vi "Test Project and Task Lists.vi"(8 "error in":errorcluster, 10 "Work Folder":path, 11 "Test Data Folder":path) -> (0 "error out":errorcluster, 2 "Report":string, 3 "Passed":bool)   [LabVIEW 2026]
doc: "Tests Project List.vi and Task List.vi on the schema-v2 sample data (Test Data\\Samples, copied into a new case folder and opened with Initialize Stores.vi). Checks: the active projects come in Sort Order with the inactive Internal left out; the project IDs are parallel to the names; the tasks of TimeTracker and of Client Website in Sort Order with the inactive Testing left out; the task named Development has a different ID in each project; an empty and an unknown Project ID give empty lists and no error.\n\nInputs: Test Data Folder (Tests\\Storage\\Test Data); Work Folder (each run works in a new case folder under it); error in. Outputs: Passed (every check passed and no error); Report (one PASS/FAIL line per check); error out.\n\nGenerated by: Claude"
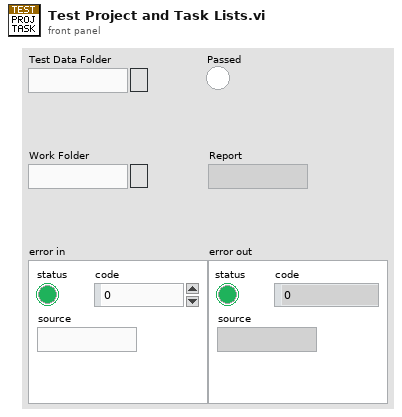
[diagram p1: front panel]
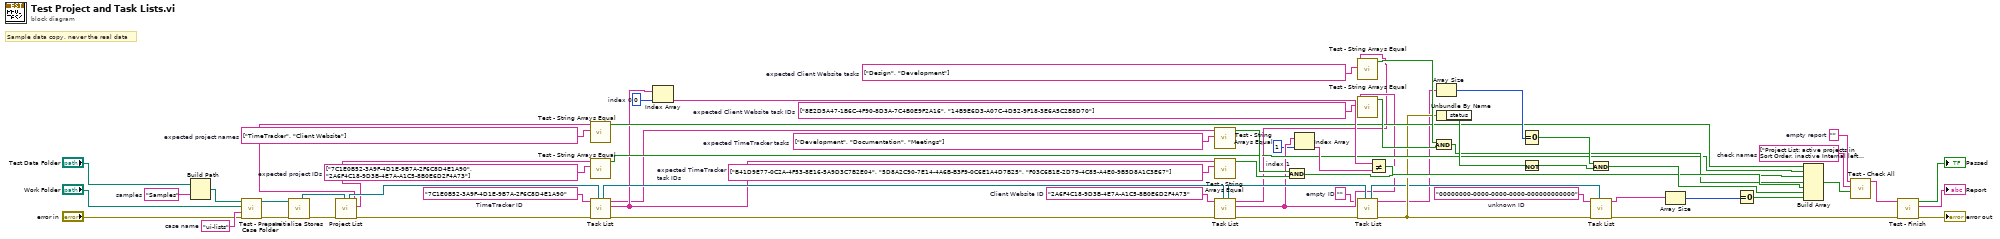
[diagram p0: block diagram]
diagram:
  w62 = string[] ["Project List: active projects in Sort Order, inactive Internal left out", "Project List: Project IDs parallel to the names", "Task List: TimeTracker tasks in Sort Order with their IDs", "Task List: Client Website tasks, inactive Testing left out, with their IDs", "Task List: Development has a different ID in each project", "Task List: empty Project ID gives an empty list and no error", "Task List: unknown Project ID gives an empty list"]  # check names
  w21 = 1  # index 1
  w20 = 0  # index 0
  w19 = string[] ["8E2D5A47-1B6C-4F90-8D3A-7C4B0E9F2A16", "14B9E6D3-A07C-4D52-9F18-3E6A5C2B8D70"]  # expected Client Website task IDs
  w18 = string[] ["Design", "Development"]  # expected Client Website tasks
  w17 = string[] ["B41D9E77-0C2A-4F53-8E16-5A9D3C7B2E04", "5D8A2C90-7E14-4A6B-B3F9-0C6E1A4D7B25", "F03C6B1E-2D79-4C85-A4E0-9B5D8A1C3E67"]  # expected TimeTracker task IDs
  w16 = string[] ["Development", "Documentation", "Meetings"]  # expected TimeTracker tasks
  w15 = string[] ["7C1E0B52-3A9F-4D1E-9B7A-2F6C8D4E1A90", "2A6F4C18-9D3B-4E7A-A1C5-8B0E6D2F4A73"]  # expected project IDs
  w14 = string[] ["TimeTracker", "Client Website"]  # expected project names
  w13 = "00000000-0000-0000-0000-000000000000"  # unknown ID
  w12 = ""  # empty ID
  w11 = "2A6F4C18-9D3B-4E7A-A1C5-8B0E6D2F4A73"  # Client Website ID
  w10 = "7C1E0B52-3A9F-4D1E-9B7A-2F6C8D4E1A90"  # TimeTracker ID
  w9 = ""  # empty report
  w8 = "ui-lists"  # case name
  w7 = "Samples"  # samples
  # "Sample data copy, never the real data"
  n1 = Build Path(base path="Test Data Folder", name or relative path=w7) -> (appended path=w22:path)
  n2 = call "Test - Prepare Case Folder.vi"("error in (no error)"="error in", "Case Name"=w8, "Work Folder"="Work Folder", "Source Folder"=w22) -> ("error out"=w24:errorcluster, "Case Folder"=w23:path)  [unwired: 6 in]
  n3 = call "Initialize Stores.vi"("error in"=w24, "Data Folder"=w23) -> ("error out"=w26:errorcluster, "Project Store out"=w25:refnum<class "Project Store.lvclass">)  [unwired: 5 in, 3 out]
  n4 = call "Project List.vi"("Project Store in"=w25, "error in"=w26) -> ("error out"=w30:errorcluster, "Project IDs"=w28:string[], "Project Names"=w27:string[], "Project Store out"=w29:refnum<class "Project Store.lvclass">)  [unwired: 6 in]
  n5 = call "Test - String Arrays Equal.vi"("Expected"=w14, "Actual"=w27) -> ("Equal?"=w44:bool)  [unwired: 8 in, 1 out]
  n6 = call "Test - String Arrays Equal.vi"("Expected"=w15, "Actual"=w28) -> ("Equal?"=w45:bool)  [unwired: 8 in, 1 out]
  n7 = call "Task List.vi"("Project Store in"=w29, "error in"=w30, "Project ID"=w10) -> ("error out"=w34:errorcluster, "Task IDs"=w32:string[], "Task Names"=w31:string[], "Project Store out"=w33:refnum<class "Project Store.lvclass">)  [unwired: 5 in]
  n8 = Index Array(array=w32, index=w20) -> (element=w52:string)
  n9 = call "Test - String Arrays Equal.vi"("Expected"=w16, "Actual"=w31) -> ("Equal?"=w46:bool)  [unwired: 8 in, 1 out]
  n10 = call "Test - String Arrays Equal.vi"("Expected"=w17, "Actual"=w32) -> ("Equal?"=w47:bool)  [unwired: 8 in, 1 out]
  n11 = call "Task List.vi"("Project Store in"=w33, "error in"=w34, "Project ID"=w11) -> ("error out"=w38:errorcluster, "Task IDs"=w36:string[], "Task Names"=w35:string[], "Project Store out"=w37:refnum<class "Project Store.lvclass">)  [unwired: 5 in]
  n12 = And(x=w46, y=w47) -> (x .and. y?=w48:bool)
  n13 = Index Array(array=w36, index=w21) -> (element=w53:string)
  n14 = call "Test - String Arrays Equal.vi"("Expected"=w18, "Actual"=w35) -> ("Equal?"=w49:bool)  [unwired: 8 in, 1 out]
  n15 = call "Test - String Arrays Equal.vi"("Expected"=w19, "Actual"=w36) -> ("Equal?"=w50:bool)  [unwired: 8 in, 1 out]
  n16 = call "Task List.vi"("Project Store in"=w37, "error in"=w38, "Project ID"=w12) -> ("error out"=w41:errorcluster, "Task Names"=w39:string[], "Project Store out"=w40:refnum<class "Project Store.lvclass">)  [unwired: 5 in, 1 out]
  n17 = Not Equal?(x=w52, y=w53) -> (x != y?=w54:bool)
  n18 = And(x=w49, y=w50) -> (x .and. y?=w51:bool)
  n19 = Array Size(array=w39) -> (size(s)=w55:i32)
  n20 = Unbundle By Name(w41) -> ("status"=w57:bool)
  n21 = Equal To 0?(x=w55) -> (x = 0?=w56:bool)
  n22 = Not(x=w57) -> (.not. x?=w58:bool)
  n23 = And(x=w56, y=w58) -> (x .and. y?=w59:bool)
  n24 = call "Task List.vi"("Project Store in"=w40, "error in"=w41, "Project ID"=w13) -> ("error out"=w43:errorcluster, "Task Names"=w42:string[])  [unwired: 5 in, 2 out]
  n25 = Array Size(array=w42) -> (size(s)=w60:i32)
  n26 = Equal To 0?(x=w60) -> (x = 0?=w61:bool)
  n27 = Build Array(w44, w45, w48, w51, w54, w59, w61) -> (w63:bool[])
  n28 = call "Test - Check All.vi"("Conditions"=w63, "Check Names"=w62, "Report in"=w9) -> ("Report out"=w64:string)  [unwired: 7 in, 1 out]
  n29 = call "Test - Finish.vi"("error in (no error)"=w43, "Report"=w64) -> ("error out"=→"error out":errorcluster, "Report out"=→"Report":string, "Passed"=→"Passed":bool)  [unwired: 7 in]
